vi "D_Upload_SDtoFMem.vi"(8 "error in (no error)":errorcluster, 9 "FMemSlotNo":u32, 10 "SDSlotNo":u32, 11 "bID":u8) -> (0 "error out":errorcluster, 3 "bID":u8, 4 "TorF":i32)   [LabVIEW 2013]
uses:
  LabVIEW2018/hpkSLMdaLV.dll
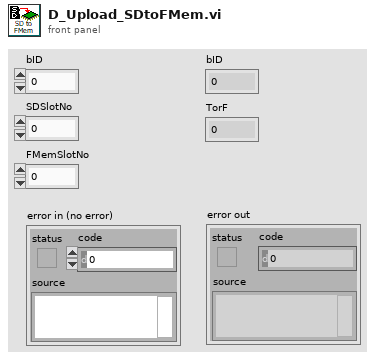
[diagram p1: front panel]
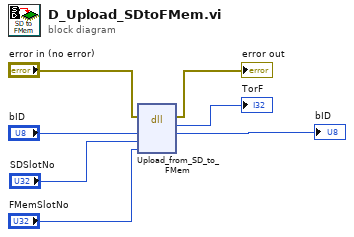
[diagram p0: block diagram]
diagram:
  n1 = dll-call lib="C:/Users/hs5921/Desktop/LabVIEW2018/hpkSLMdaLV.dll" fn="Upload_from_SD_to_FMem"(error in="error in (no error)", "bID"="bID", "SDSlotNo"="SDSlotNo", "FMemSlotNo"="FMemSlotNo") -> (error out=→"error out":errorcluster, "返り値タイプ"=→"TorF":i32, "bID"=→"bID":u8)  [unwired: 4 in, 1 out]
